vi "RDV-getNames.vi"(11 "RDV-Reflection_Data_viewer in":refnum<class "RDV-Reflection_Data_viewer.lvclass">) -> (0 "Sets of data":string[](array[string]), 1 "other names":string[](array[string]), 2 "Ignore Names":string[](array[string]))   [LabVIEW 2020, in "RDV-Reflection_Data_viewer.lvclass"]
doc: "Returns the names of the data sets, the other names and the ignore names held by the viewer."
uses:
  RDV-Reflection_Data_viewer.lvclass
  Computation/RDC-perm_calc_type.ctl
  RDV-Reflection_Data_viewer.lvclass/RDV-Reflection_Data_viewer.ctl
  Computation/RDC-Reflection_Data_Computation.lvlib
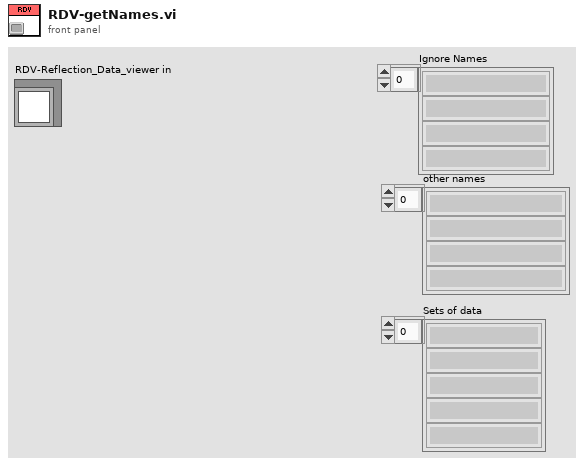
[diagram p1: front panel]
types:
  T1 = typedef "RDC-Reflection_Data_Computation.lvlib/RDC-perm_calc_type.ctl" = enum16{"Basic", "Capacative", "Advance", "Bilinear", "Size"}
  T2 = typedef "RDV-Reflection_Data_viewer.lvclass/RDV-UPDATE_IGNORE_LIST.ctl" = string[]
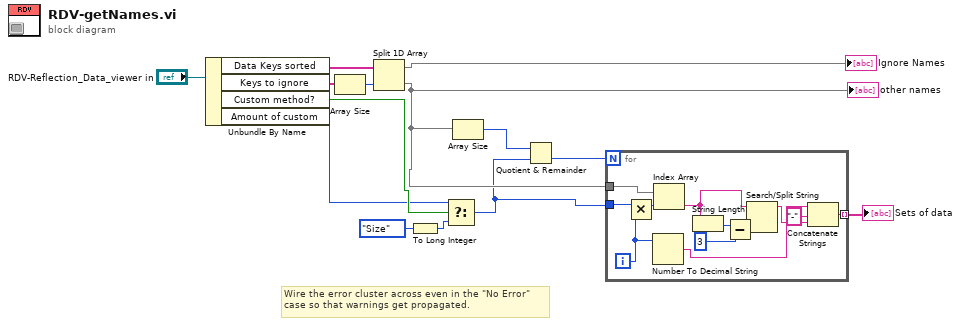
[diagram p0: block diagram]
diagram:
  # "Wire the error cluster across even in the \"No Error\"\ncase so that warnings get propagated."
  n1 = Unbundle By Name("RDV-Reflection_Data_viewer in") -> ("Data Keys sorted"=w10:string[], "Keys to ignore"=w11:T2, "Custom method?"=w2:bool, "Amount of custom"=w1:i32)
  n2 = Array Size(array=w11) -> (size(s)=w12:i32)
  n3 = Split 1D Array(array=w10, index=w12) -> (first subarray=→"Ignore Names":string[], second subarray=w7:string[])
  "other names" <- w7
  n4 = To Long Integer(number=RDC-perm_calc_type."Size" ("Perm calc type")) -> (32bit integer=w4:i32)
  n5 = Select(t=w1, s=w2, f=w4) -> (s? t:f=w3:i32)
  n6 = Array Size(array=w7) -> (size(s)=w6:i32)
  n7 = Quotient & Remainder(x=w6, y=w3) -> (floor(x/y)=w5:i32)  [unwired: 1 out]
  n8 = for {
    N: w5 -> [_]
    tunnel: w7 -> [w26]
    tunnel: w3 -> [w25]
    tunnel: [w18] -> w8 mode=indexing
    i -> [w17]
    n9 = Multiply(x=w25, y=w17) -> (x*y=w24:i32)
    n10 = Number To Decimal String(number=w17) -> (decimal integer string=w16:string)  [unwired: 1 in]
    n11 = Index Array(array=w26, index=w24) -> (element=w23:string)
    n12 = String Length(string=w23) -> (length=w22:i32)
    n13 = Subtract(x=w22, y=3) -> (x-y=w20:i32)
    n14 = Search/Split String(string=w23, offset (0)=w20) -> (substring before match=w19:string)  [unwired: 1 in, 2 out]
    n15 = Concatenate Strings(w16, "-" ("string"), w19) -> (w18:string)
  }
  "Sets of data" <- w8
